vi "Resume.vi"(6 "nargs":i32, 10 "error in (no error)":errorcluster, 11 "Lua in":refnum<class "Lua.lvclass">) -> (1 "done?":bool, 2 "error out":errorcluster, 3 "Lua out":refnum<class "Lua.lvclass">, 4 "nresults":i32)   [LabVIEW 2020, in "Lua for LabVIEW.lvlib" / "Lua.lvclass"]
doc: "Starts and resumes a coroutine in the given thread L.\n\nTo start a coroutine, you push onto the thread stack the main function plus any arguments; then you call lua_resume, with nargs being the number of arguments. This call returns when the coroutine suspends or finishes its execution. When it returns, the stack contains all values passed to lua_yield, or all values returned by the body function. lua_resume returns LUA_YIELD if the coroutine yields, LUA_OK if the coroutine finishes its execution without errors, or an error code in case of errors (see lua_pcall).\n\nIn case of errors, the stack is not unwound, so you can use the debug API over it. The error object is on the top of the stack.\n\nTo resume a coroutine, you remove any results from the last lua_yield, put on its stack only the values to be passed as results from yield, and then call lua_resume.\n\nThe parameter from represents the coroutine that is resuming L. If there is no such coroutine, this parameter can be NULL."
uses:
  Lua.lvclass
  Lua.lvclass/Lua.ctl
  lib/lua.dll/lua_thread_status.ctl
  lib/lua.dll/lua_types.ctl
  lib/lua.dll/lua_tolstring.vi
  lib/lua.dll/lua_pop.vi
  lib/lua.dll/lua_settop.vi
  lib/lua.dll/lua.dll.lvlib
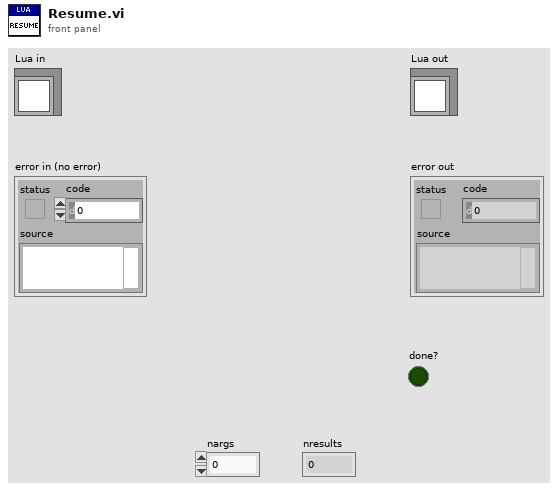
[diagram p1: front panel]
types:
  T1 = typedef "lua.dll.lvlib/lua_thread_status.ctl" = enum8{"LUA_OK", "LUA_YIELD", "LUA_ERRRUN", "LUA_ERRSYNTAX", "LUA_ERRMEM", "LUA_ERRERR"}
  T2 = typedef "lua.dll.lvlib/lua_types.ctl" = i32
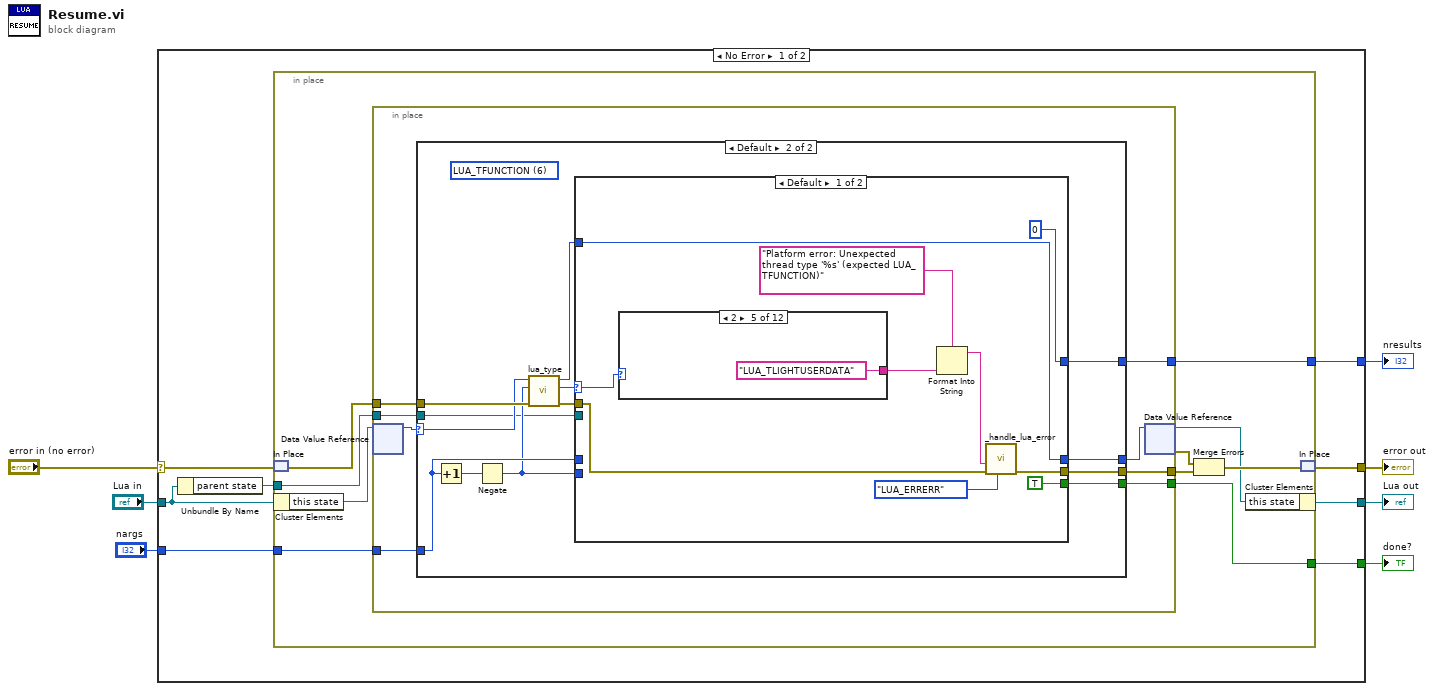
[diagram p0: block diagram]
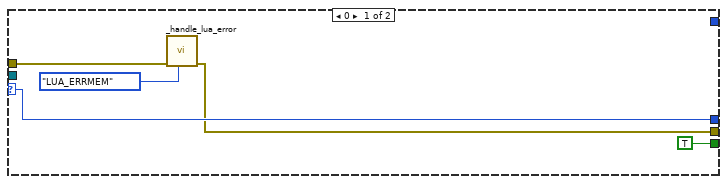
[diagram p2: hidden frame]
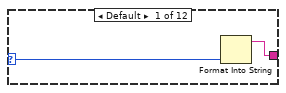
[diagram p3: hidden frame]
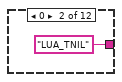
[diagram p4: hidden frame]
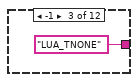
[diagram p5: hidden frame]
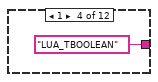
[diagram p6: hidden frame]
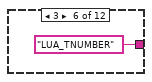
[diagram p7: hidden frame]
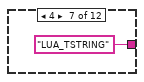
[diagram p8: hidden frame]
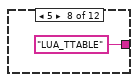
[diagram p9: hidden frame]
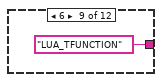
[diagram p10: hidden frame]
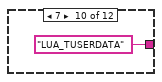
[diagram p11: hidden frame]
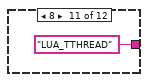
[diagram p12: hidden frame]
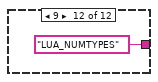
[diagram p13: hidden frame]
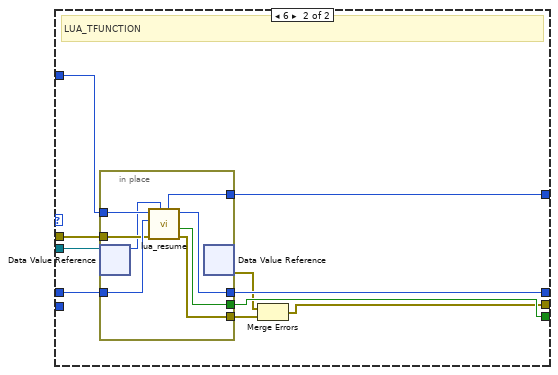
[diagram p14: hidden frame]
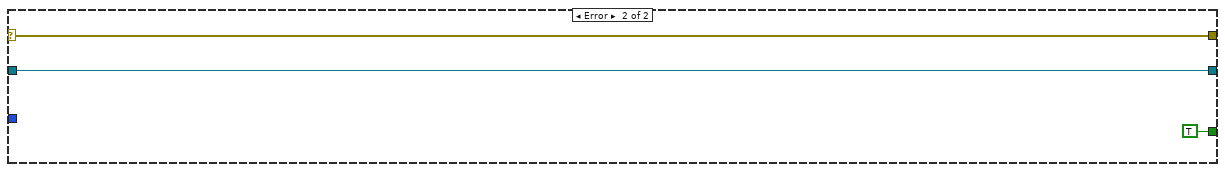
[diagram p15: hidden frame]
diagram:
  n1 = case shown="No Error" "error in (no error)" {
    selector: "error in (no error)" -> [w13 w95]
    tunnel: [w14 w95] -> w4
    tunnel: [w15 w94] -> w7
    tunnel: "Lua in" -> [w9 w94]
    tunnel: "nargs" -> [w12 _]
    tunnel: [w11 _] -> w2
    tunnel: [w10 TRUE ("done?")] -> w1
    frame No Error {
      n2 = Unbundle By Name(w9) -> ("parent state"=w8:refnum<data-value>)
      n3 = in-place {
        in-place-border: w12 -> [w24]
        in-place-border: [w23] -> w11
        in-place-border: [w22] -> w10
        in-place-border: w8 -> [w21]
        n4 = in-place-match #1(w13) -> (w25:errorcluster)
        n5 = in-place-cluster #2(w9) -> ("this state"=w19:refnum<data-value>)
        n6 = in-place {
          in-place-border: w25 -> [w33]
          in-place-border: w24 -> [w32]
          in-place-border: [w31] -> w23
          in-place-border: [w30] -> w22
          in-place-border: w21 -> [w29]
          in-place-border: [w26] -> w16
          n7 = in-place-dvr #3(w19) -> (w28:u64)  [unwired: 1 out]
          n8 = case shown="Default" w28 {
            selector: w28 -> [w38 w43]
            tunnel: [w38 w51] -> w27
            tunnel: w33 -> [w36 w46]
            tunnel: [w37 w49] -> w26
            tunnel: w32 -> [_ w47]
            tunnel: [_ w48] -> w31
            tunnel: [TRUE ("done?") w50] -> w30
            tunnel: w29 -> [_ w39]
            frame 0 {
              n9 = call "_handle_lua_error.vi"("lua status"=lua_thread_status."LUA_ERRMEM", "error in (no error)"=w36) -> ("error out"=w37:errorcluster)  [unwired: 9 in]
            }
            frame Default {
              (unwired) T2 6 items=["LUA_TNONE"=-1, "LUA_TNIL"=0, "LUA_TBOOLEAN"=1, "LUA_TLIGHTUSERDATA"=2, "LUA_TNUMBER"=3, "LUA_TSTRING"=4, "LUA_TTABLE"=5, "LUA_TFUNCTION"=6, "LUA_TUSERDATA"=7, "LUA_TTHREAD"=8, "LUA_NUMTYPES"=9] ("lua type")
              n10 = Increment(x=w47) -> (x+1=w45:i32)
              n11 = Negate(x=w45) -> (-x=w41:i32)
              n12 = call "lua_type.vi"("error in (no error)"=w46, "index"=w41, "lua_state_p"=w43) -> ("error out"=w40:errorcluster, "lua type"=w44:T2, "lua_state_p out"=w42:u64)  [unwired: 6 in]
              n13 = case shown="Default" w44 {
                selector: w44 -> [w53 _]
                tunnel: [w59 w82] -> w51
                tunnel: [TRUE ("done?") w84] -> w50
                tunnel: [w58 w75] -> w49
                tunnel: [0 ("nresults") w80] -> w48
                tunnel: w42 -> [w59 w81]
                tunnel: w47 -> [_ w83]
                tunnel: w40 -> [w57 w79]
                tunnel: w41 -> [_ _]
                tunnel: w39 -> [_ w78]
                frame Default {
                  n14 = case shown="2" w53 {
                    selector: w53 -> [w63 _ _ _ _ _ _ _ _ _ _ _]
                    tunnel: [w62 "LUA_TNIL" "LUA_TNONE" "LUA_TBOOLEAN" "LUA_TLIGHTUSERDATA" "LUA_TNUMBER" "LUA_TSTRING" "LUA_TTABLE" "LUA_TFUNCTION" "LUA_TUSERDATA" "LUA_TTHREAD" "LUA_NUMTYPES"] -> w52
                    frame Default {
                      n15 = Format Into String(w63) -> (resulting string=w62:string)  [unwired: 3 in, 1 out]
                    }
                    frame 0 {
                    }
                    frame -1 {
                    }
                    frame 1 {
                    }
                    frame 2 {
                    }
                    frame 3 {
                    }
                    frame 4 {
                    }
                    frame 5 {
                    }
                    frame 6 {
                    }
                    frame 7 {
                    }
                    frame 8 {
                    }
                    frame 9 {
                    }
                  }
                  n16 = Format Into String(format string="Platform error: Unexpected thread type '%s' (expected LUA_TFUNCTION)" ("error string"), w52) -> (resulting string=w55:string)  [unwired: 2 in, 1 out]
                  n17 = call "_handle_lua_error.vi"("lua status"=lua_thread_status."LUA_ERRERR", "error in (no error)"=w57, "error string"=w55) -> ("error out"=w58:errorcluster)  [unwired: 8 in]
                }
                frame 6 {
                  # "LUA_TFUNCTION"
                  n18 = in-place {
                    in-place-border: [w92] -> w84
                    in-place-border: w83 -> [w91]
                    in-place-border: [w90] -> w82
                    in-place-border: w81 -> [w89]
                    in-place-border: [w88] -> w76
                    in-place-border: [w87] -> w80
                    in-place-border: w79 -> [w86]
                    n19 = in-place-dvr #4(w78) -> (w85:u64)  [unwired: 1 out]
                    n20 = call "lua_resume.vi"("from_p"=w85, "error in (no error)"=w86, "nargs"=w91, "lua_state_p"=w89) -> ("error out"=w88:errorcluster, "done?"=w92:bool, "lua_state_p out"=w90:u64, "nresults"=w87:i32)  [unwired: 4 in]
                    n21 = in-place-dvr #4() -> (w77:errorcluster)  [unwired: 1 in, 1 out]
                  }
                  n22 = Merge Errors(w77, w76) -> (w75:errorcluster)
                }
              }
            }
          }
          n23 = in-place-dvr #3(w27) -> (w18:refnum<data-value>, w17:errorcluster)
        }
        n24 = Merge Errors(w17, w16) -> (w20:errorcluster)
        n25 = in-place-cluster #2("this state"=w18) -> (w15:refnum<class "Lua.lvclass">)
        n26 = in-place-match #1(w20) -> (w14:errorcluster)
      }
    }
    frame Error {
    }
  }
  "error out" <- w4
  "Lua out" <- w7
  "nresults" <- w2
  "done?" <- w1
